vi "Assemble BoundViewManager.vi"(4 "Default View Name (\"\"=None)":string, 6 "Startup View Name (\"\"=None)":string, 7 "Insert View on Value Change Only? (T)":bool=TRUE, 8 "Selector String Name":string, 9 "Viewable Names":string[](array[string]), 10 "Bound Viewables":refnum<class "IViewable.lvclass">[](array[class])) -> (3 "BoundViewManager Out":refnum<class "BoundViewManager.lvclass">)   [LabVIEW 2018, in "MVA Framework.lvlib" / "BoundViewManager.lvlib" / "BoundViewManager.lvclass"]
doc: "组装绑定视图管理器"
uses:
  BoundViewManager.lvclass
  modules/mva-viewable/Source/IViewManager/IViewManager/IViewManager.lvclass
  modules/mva-viewable/Source/IViewable/IViewable/IViewable.lvclass
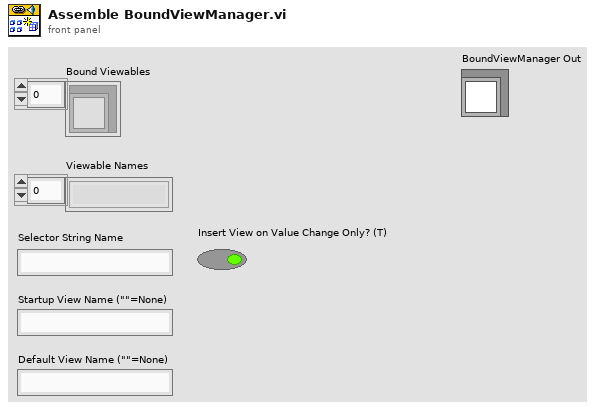
[diagram p1: front panel]
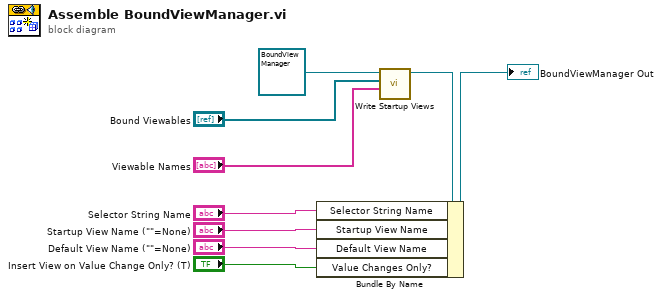
[diagram p0: block diagram]
diagram:
  n1 = call "Write Startup Views.vi"("View Labels"="Viewable Names", "Startup Views"="Bound Viewables", "IViewManager in"=refnum<class "BoundViewManager.lvclass"> refnum ("BoundViewManager")) -> ("IViewManager out"=w6:refnum<class "BoundViewManager.lvclass">)  [unwired: 8 in]
  n2 = Bundle By Name(cluster=w6, "Selector String Name"="Selector String Name", "Startup View Name"="Startup View Name (\"\"=None)", "Default View Name"="Default View Name (\"\"=None)", "Value Changes Only?"="Insert View on Value Change Only? (T)") -> (→"BoundViewManager Out":refnum<class "BoundViewManager.lvclass">)
